vi "set TDF On.vi"(8 "error in (no error)":errorcluster caption="에러 입력(에러 없음)", 9 "On?":bool, 10 "File Name":string, 11 "FSV-40N 입력":refnum<class "FSV-40N.lvclass">) -> (0 "error out":errorcluster caption="에러 출력", 3 "FSV-40N 출력":refnum<class "FSV-40N.lvclass">)   [LabVIEW 2023, in "Spectrum Analyzer.lvlib" / "FSV-40N.lvclass"]
uses:
  FSV-40N.lvclass
  FSV-40N.lvclass/FSV-40N.ctl
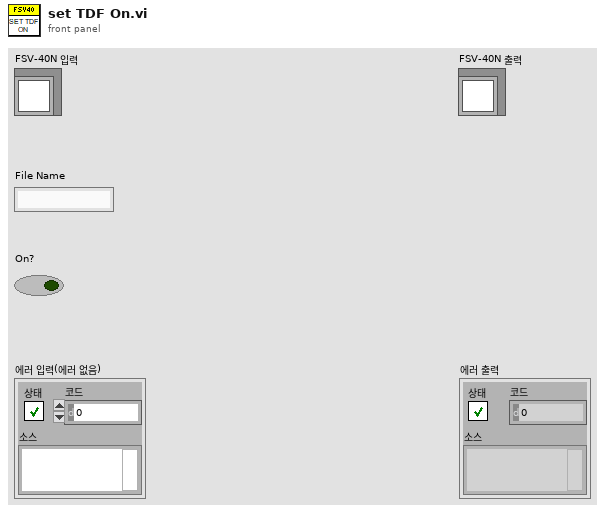
[diagram p1: front panel]
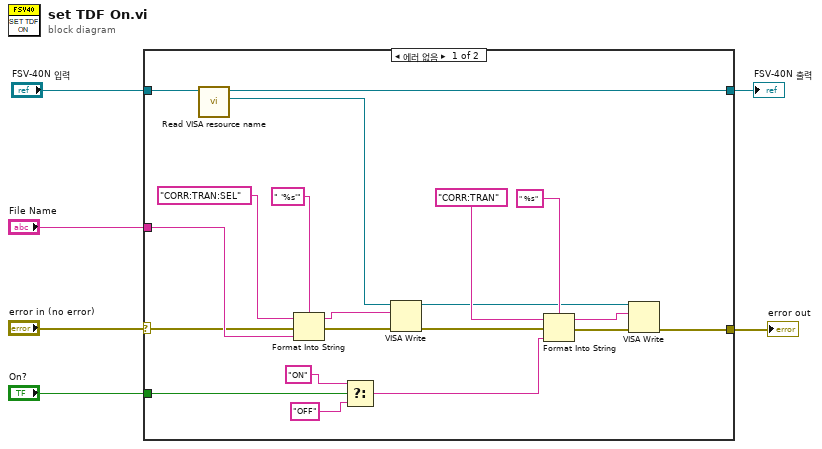
[diagram p0: block diagram]
diagram:
  n1 = case shown="에러 없음" "error in (no error)" {
    selector: "error in (no error)" -> [w22 w27]
    tunnel: "FSV-40N 입력" -> [w26 w28]
    tunnel: "File Name" -> [w23 _]
    tunnel: "On?" -> [w21 _]
    tunnel: [w9 w28] -> w2
    tunnel: [w8 w27] -> w1
    frame No Error {
      n2 = call "Read VISA resource name.vi"("FSV-40N in"=w26) -> ("VISA resource name"=w15:refnum<visa-resource-name>, "FSV-40N out"=w9:refnum<class "FSV-40N.lvclass">)  [unwired: 8 in, 1 out]
      n3 = Format Into String(format string=" '%s'", initial string="CORR:TRAN:SEL", error in=w22, w23) -> (resulting string=w14:string, error out=w13:errorcluster)
      n4 = Select(t="ON", s=w21, f="OFF") -> (s? t:f=w16:string)
      n5 = VISA Write(VISA resource name=w15, write buffer=w14, error in (no error)=w13) -> (VISA resource name out=w10:refnum<visa-resource-name>, error out=w12:errorcluster)  [unwired: 1 out]
      n6 = Format Into String(format string=" %s", initial string="CORR:TRAN" ("초기 문자열"), error in=w12, w16) -> (resulting string=w7:string, error out=w11:errorcluster)
      n7 = VISA Write(VISA resource name=w10, write buffer=w7, error in (no error)=w11) -> (error out=w8:errorcluster)  [unwired: 2 out]
    }
    frame Error {
    }
  }
  "error out" <- w1
  "FSV-40N 출력" <- w2
